vi "fetch CHP Power Value.vi"(8 "error in (no error)":errorcluster, 11 "Keysight 9020A in":refnum<class "Keysight 9020A.lvclass">) -> (0 "error out":errorcluster, 2 "Channel Power":dbl, 3 "Keysight 9020A out":refnum<class "Keysight 9020A.lvclass">)   [LabVIEW 2023, in "Spectrum Analyzer.lvlib" / "Keysight 9020A.lvclass"]
uses:
  Keysight 9020A.lvclass
  Keysight 9020A.lvclass/Keysight 9020A.ctl
  Spectrum Analyzer.lvlib
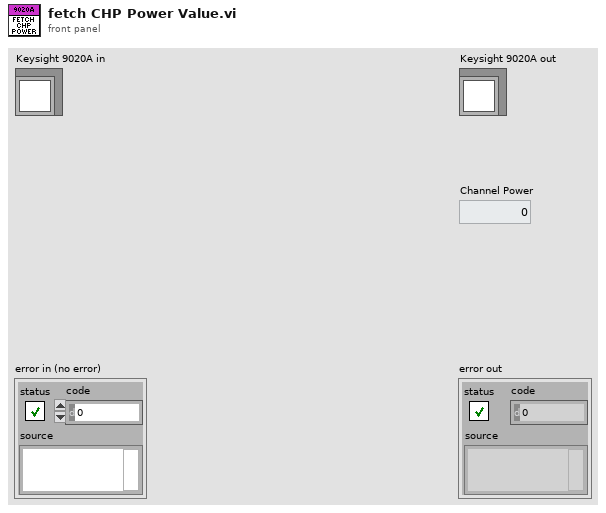
[diagram p1: front panel]
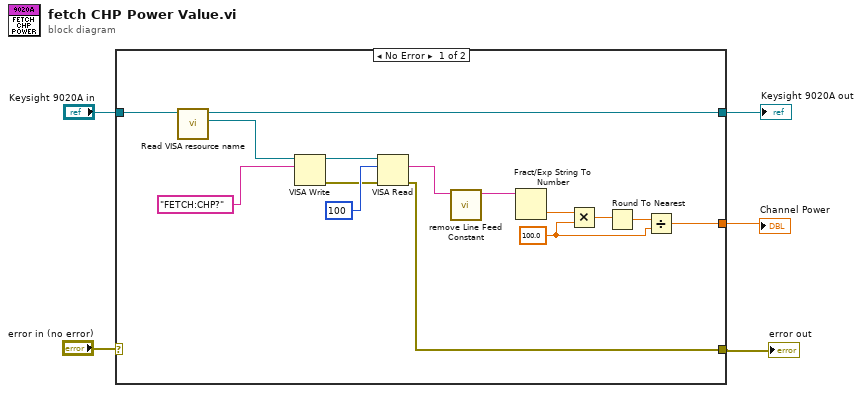
[diagram p0: block diagram]
diagram:
  n1 = case shown="No Error" "error in (no error)" {
    selector: "error in (no error)" -> [_ w21]
    tunnel: "Keysight 9020A in" -> [w18 w22]
    tunnel: [w20 w22] -> w4
    tunnel: [w7 w21] -> w2
    tunnel: [w6 _] -> w1
    frame No Error {
      w9 = 100.0 ("y")
      n2 = call "Read VISA resource name.vi"("Keysight 9020A in"=w18) -> ("VISA resource name"=w19:refnum<visa-resource-name>, "Keysight 9020A out"=w20:refnum<class "Keysight 9020A.lvclass">)  [unwired: 8 in, 1 out]
      n3 = VISA Write(VISA resource name=w19, write buffer="FETCH:CHP?") -> (VISA resource name out=w15:refnum<visa-resource-name>, error out=w14:errorcluster)  [unwired: 1 in, 1 out]
      n4 = VISA Read(VISA resource name=w15, byte count=u32 100, error in (no error)=w14) -> (read buffer=w13:string, error out=w7:errorcluster)  [unwired: 2 out]
      n5 = call "remove Line Feed Constant.vi"("Input String"=w13) -> ("Line Feed Removed String"=w8:string)  [unwired: 10 in]
      n6 = Fract/Exp String To Number(string=w8) -> (number=w11:dbl)  [unwired: 3 in, 1 out]
      n7 = Multiply(x=w11, y=w9) -> (x*y=w12:dbl)
      n8 = Round To Nearest(number=w12) -> (nearest integer value=w10:dbl)
      n9 = Divide(x=w10, y=w9) -> (x/y=w6:dbl)
    }
    frame Error {
    }
  }
  "error out" <- w2
  "Keysight 9020A out" <- w4
  "Channel Power" <- w1
